vi "Unflatten Buffer Configuration.vi"(11 "Flattened Configuration":u8[](array[numeric]) format="%.0x") -> (3 "Buffer Configuration":T1)   [LabVIEW 2021, in "CIF_CIPC_Chn.lvclass"]
uses:
  CIF_CIPC_Chn.lvclass
  Typedef/Buffer Configuration Data.ctl
  <vilib>/CIF Foundation/CIF CIPC/TypeDefs/Backpressure References.ctl
  <vilib>/CIF Foundation/CIF CIPC/TypeDefs/Backpressure Names.ctl
  CIF_CIPC_Chn.lvclass/CIF_CIPC_Chn.ctl
  <vilib>/CIF Foundation/CIF Utilities/DataTypes/DataTypes_CIF_U.lvlib
  <vilib>/CIF Foundation/CIF CIPC/CIF_NI_CIPC.lvlib
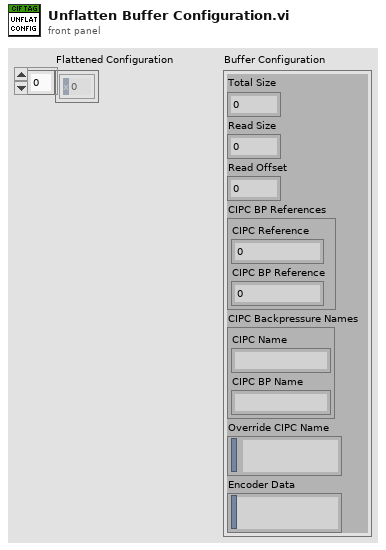
[diagram p1: front panel]
types:
  T1 = typedef "CIF_CIPC_Chn.lvclass/Buffer Configuration Data.ctl" = cluster{"Total Size":u32, "Read Size":u32, "Read Offset":u32, "CIPC BP References":T2, "CIPC Backpressure Names":T3, "Override CIPC Name":string, "Encoder Data":string}
  T2 = typedef "CIF_NI_CIPC.lvlib/Backpressure References.ctl" = cluster{"CIPC Reference":u64, "CIPC BP Reference":u64}
  T3 = typedef "CIF_NI_CIPC.lvlib/Backpressure Names.ctl" = cluster{"CIPC Name":string, "CIPC BP Name":string}
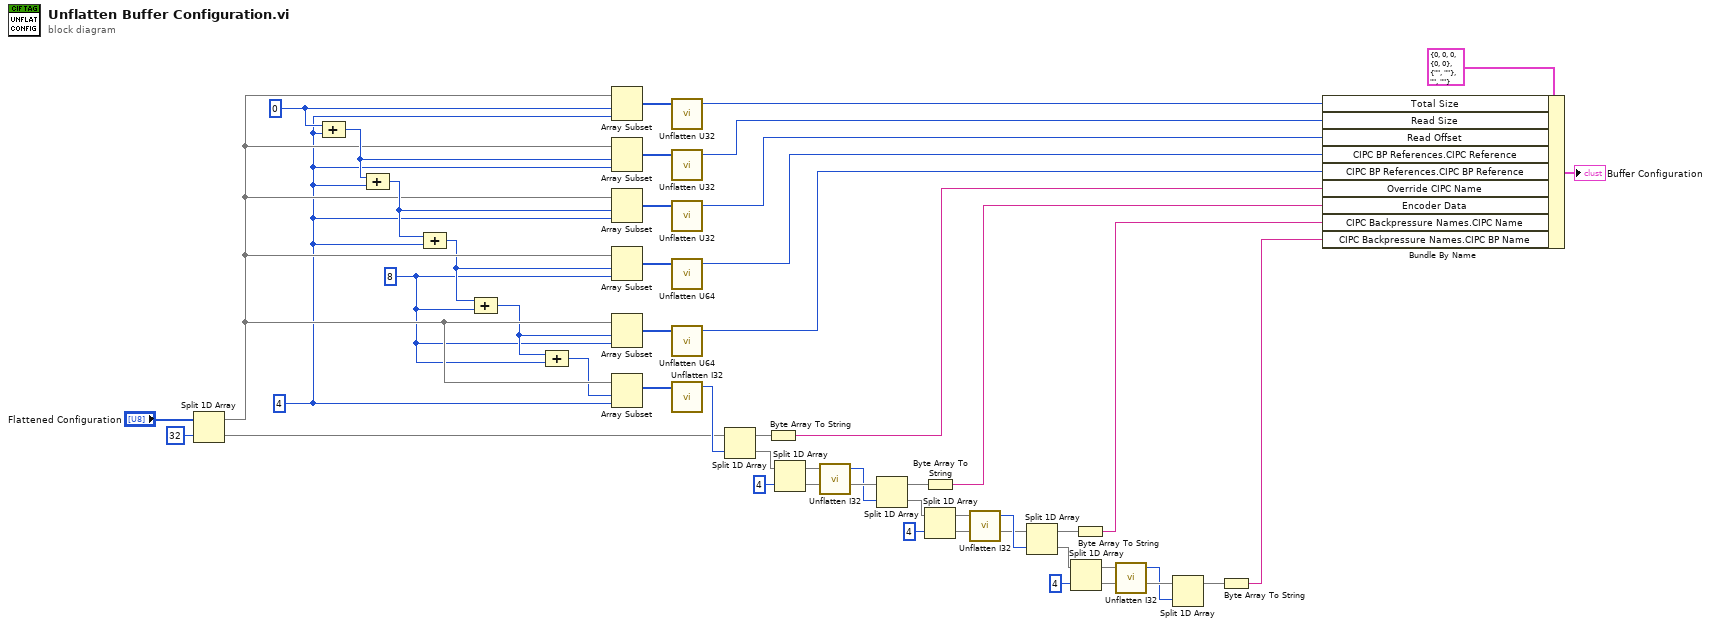
[diagram p0: block diagram]
diagram:
  w15 = 8 ("length")
  w19 = 4 ("length")
  w47 = 0 ("index")
  n1 = Split 1D Array(array="Flattened Configuration", index=32) -> (first subarray=w23:u8[], second subarray=w35:u8[])
  n2 = Compound Arithmetic op=unknown(w47, w19) -> (w46:i32)
  n3 = Compound Arithmetic op=unknown(w46, w19) -> (w37:i32)
  n4 = Compound Arithmetic op=unknown(w37, w19) -> (w22:i32)
  n5 = Compound Arithmetic op=unknown(w22, w15) -> (w21:i32)
  n6 = Compound Arithmetic op=unknown(w21, w15) -> (w20:i32)
  n7 = Array Subset(array=w23, index=w47, length=w19) -> (w43:u8[])
  n8 = Array Subset(array=w23, index=w46, length=w19) -> (w44:u8[])
  n9 = Array Subset(array=w23, index=w37, length=w19) -> (w45:u8[])
  n10 = Array Subset(array=w23, index=w22, length=w15) -> (w25:u8[])
  n11 = Array Subset(array=w23, index=w21, length=w15) -> (w24:u8[])
  n12 = Array Subset(array=w23, index=w20, length=w19) -> (w18:u8[])
  n13 = call <vilib>:"Unflatten U32.vi"("Flat Data"=w43) -> ("U32"=w42:u32)  [unwired: 4 in]
  n14 = call <vilib>:"Unflatten U32.vi"("Flat Data"=w44) -> ("U32"=w41:u32)  [unwired: 4 in]
  n15 = call <vilib>:"Unflatten U32.vi"("Flat Data"=w45) -> ("U32"=w40:u32)  [unwired: 4 in]
  n16 = call <vilib>:"Unflatten U64.vi"("Flat Data"=w25) -> ("U64"=w17:u64)  [unwired: 4 in]
  n17 = call <vilib>:"Unflatten U64.vi"("Flat Data"=w24) -> ("U64"=w16:u64)  [unwired: 4 in]
  n18 = call <vilib>:"Unflatten I32.vi"("Flat Data"=w18) -> ("I32"=w36:i32)  [unwired: 4 in]
  n19 = Split 1D Array(array=w35, index=w36) -> (first subarray=w34:u8[], second subarray=w32:u8[])
  n20 = Byte Array To String(unsigned byte array=w34) -> (string=w33:string)
  n21 = Split 1D Array(array=w32, index=4) -> (first subarray=w29:u8[], second subarray=w28:u8[])
  n22 = call <vilib>:"Unflatten I32.vi"("Flat Data"=w29) -> ("I32"=w27:i32)  [unwired: 4 in]
  n23 = Split 1D Array(array=w28, index=w27) -> (first subarray=w26:u8[], second subarray=w9:u8[])
  n24 = Byte Array To String(unsigned byte array=w26) -> (string=w30:string)
  n25 = Split 1D Array(array=w9, index=4) -> (first subarray=w11:u8[], second subarray=w12:u8[])
  n26 = call <vilib>:"Unflatten I32.vi"("Flat Data"=w11) -> ("I32"=w13:i32)  [unwired: 4 in]
  n27 = Split 1D Array(array=w12, index=w13) -> (first subarray=w14:u8[], second subarray=w3:u8[])
  n28 = Split 1D Array(array=w3, index=4) -> (first subarray=w7:u8[], second subarray=w6:u8[])
  n29 = Byte Array To String(unsigned byte array=w14) -> (string=w2:string)
  n30 = call <vilib>:"Unflatten I32.vi"("Flat Data"=w7) -> ("I32"=w5:i32)  [unwired: 4 in]
  n31 = Split 1D Array(array=w6, index=w5) -> (first subarray=w4:u8[])  [unwired: 1 out]
  n32 = Byte Array To String(unsigned byte array=w4) -> (string=w1:string)
  n33 = Bundle By Name(cluster=T1 {"Total Size"=0, "Read Size"=0, "Read Offset"=0, "CIPC BP References"={"CIPC Reference"=0, "CIPC BP Reference"=0}, "CIPC Backpressure Names"={"CIPC Name"="", "CIPC BP Name"=""}, "Override CIPC Name"="", "Encoder Data"=""} ("Buffer Configuration"), "Total Size"=w42, "Read Size"=w41, "Read Offset"=w40, "CIPC BP References.CIPC Reference"=w17, "CIPC BP References.CIPC BP Reference"=w16, "Override CIPC Name"=w33, "Encoder Data"=w30, "CIPC Backpressure Names.CIPC Name"=w2, "CIPC Backpressure Names.CIPC BP Name"=w1) -> (→"Buffer Configuration":T1)
